vi "Execute.vi"(8 "error in (no error)":errorcluster, 11 "Node in":refnum<class "bt_Decorator.lvclass">) -> (0 "error out":errorcluster, 1 "Status":T1, 3 "Node out":refnum<class "bt_Decorator.lvclass">)   [LabVIEW 2021, in "BT.lvlib" / "bt_Decorator.lvclass"]
uses:
  bt_Decorator.lvclass
  abs_Node/Status.ctl
  bt_Decorator.lvclass/bt_Decorator.ctl
  abs_Node/bt_Node.lvclass
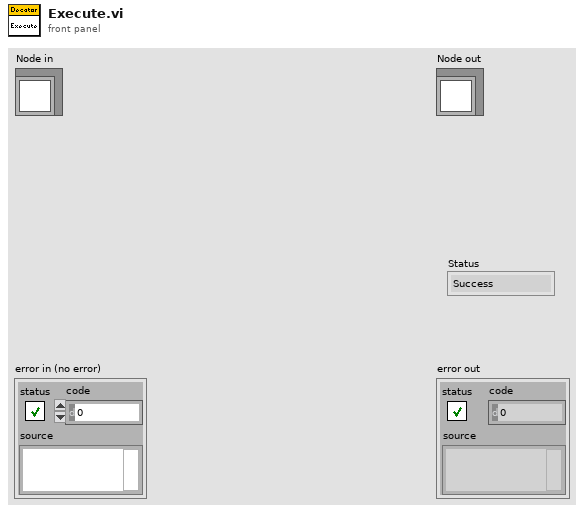
[diagram p1: front panel]
types:
  T1 = typedef "BT.lvlib/bt_Node.lvclass/Status.ctl" = enum16{"Success", "Failure", "Running"}
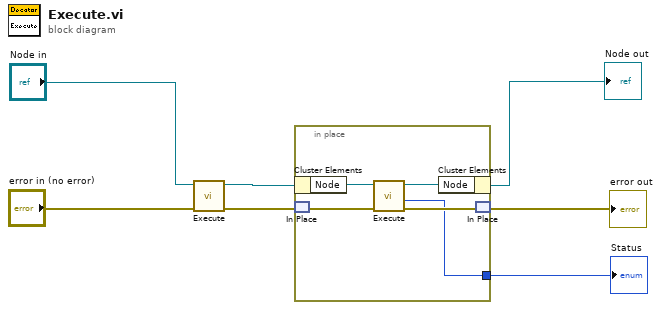
[diagram p0: block diagram]
diagram:
  n1 = call-parent "Execute.vi"("error in (no error)"="error in (no error)", "Node in"="Node in") -> ("error out"=w1:errorcluster, "Node out"=w2:refnum<class "bt_Decorator.lvclass">)  [unwired: 7 in, 1 out]
  n2 = in-place {
    in-place-border: [w8] -> w3
    n3 = in-place-cluster #1(w2) -> ("Node"=w12:refnum<class "bt_Node.lvclass">)
    n4 = in-place-match #2(w1) -> (w10:errorcluster)
    n5 = call-dynamic "Execute.vi"("error in (no error)"=w10, "Node in"=w12) -> ("error out"=w9:errorcluster, "Status"=w8:T1, "Node out"=w11:refnum<class "bt_Node.lvclass">)  [unwired: 7 in]
    n6 = in-place-cluster #1("Node"=w11) -> (→"Node out":refnum<class "bt_Decorator.lvclass">)
    n7 = in-place-match #2(w9) -> (→"error out":errorcluster)
  }
  "Status" <- w3
